vi "PromptUserWithDefault.vi"(7 "is Category?":bool, 9 "Recommended Name (\"\": None)":string, 10 "Structure Type":T1, 11 "Section":string) -> (1 "OK":bool, 2 "NewTag 2":string caption="NewTag")   [LabVIEW 2020]
uses:
  StructureTypes.ctl
  <userlib>/_OpenG.lib/appcontrol/appcontrol.llb/openg_application_control.lvlib
panel:
  in  "New Frame Name":string caption="NewTag"
  out "error out":errorcluster
  in  "error in (no error)":errorcluster
  out "String":string="Enter new case name or hit 'Cancel'."
  in  "Enable":bool=TRUE
  in  "Cancel":bool
  in  "OK2":bool
  in  "OK1":bool
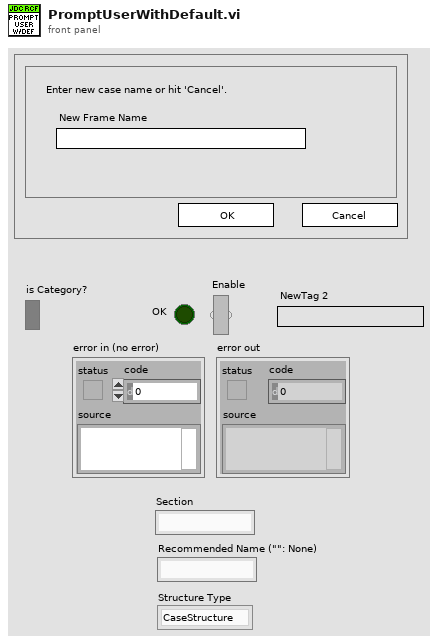
[diagram p1: front panel]
types:
  T1 = typedef "StructureTypes.ctl" = enum16{"CaseStructure", "EventStructure"}
  T2 = cluster{"Selection Start":u32, "Selection End":u32}
  T3 = cluster{"Input Name":string, "Input Data Type":i32}[]
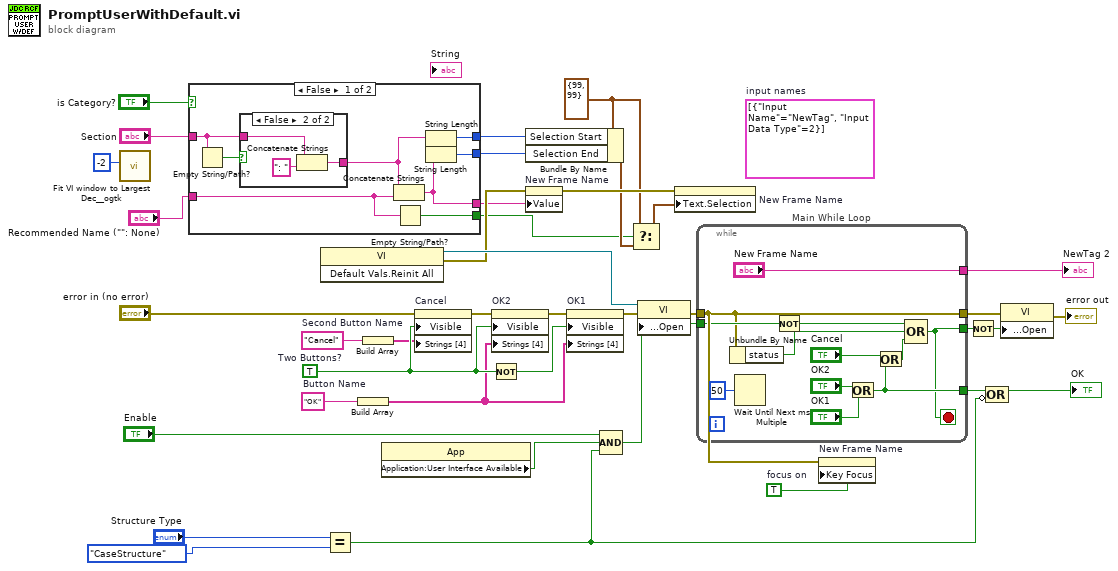
[diagram p0: block diagram]
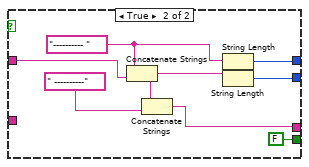
[diagram p3: hidden frame]
diagram:
  w6 = T2 {"Selection Start"=99, "Selection End"=99} ("Text.Selection")
  w23 = TRUE  # focus on
  (unwired) T3 [{"Input Name"="NewTag", "Input Data Type"=2}]  # input names
  w32 = "Cancel"  # Second Button Name
  w30 = "OK"  # Button Name
  w39 = TRUE  # Two Buttons?
  n1 = call <userlib>:"Fit VI window to Largest Dec__ogtk.vi"("border spacing (2 px)"=-2) -> ()  [unwired: 5 in, 2 out]
  n2 = case shown="False" "is Category?" {
    tunnel: "Section" -> [w41 w57]
    tunnel: "Recommended Name (\"\": None)" -> [w43 _]
    tunnel: [w46 w52] -> w7
    tunnel: [w45 w55] -> w4
    tunnel: [w44 w59] -> w3
    tunnel: [w42 FALSE] -> w1
    frame False {
      n3 = Empty String/Path?(string/path=w41) -> (empty?=w40:bool)
      n4 = case shown="False" w40 {
        tunnel: [w48 w50] -> w47
        tunnel: w41 -> [w48 w49]
        frame True {
        }
        frame False {
          n5 = Concatenate Strings(w49, ": " ("string")) -> (w50:string)
        }
      }
      n6 = Concatenate Strings(w47, w43) -> (w46:string)
      n7 = Empty String/Path?(string/path=w43) -> (empty?=w42:bool)
      n8 = String Length(string=w47) -> (length=w45:i32)
      n9 = String Length(string=w46) -> (length=w44:i32)
    }
    frame True {
      w54 = "---------- " ("Section")
      n10 = Concatenate Strings(w54, w57) -> (w53:string)
      n11 = Concatenate Strings(w53, " ----------" ("Section")) -> (w52:string)
      n12 = String Length(string=w54) -> (length=w55:i32)
      n13 = String Length(string=w53) -> (length=w59:i32)
    }
  }
  n14 = invoke class="VI" method="Default Vals.Reinit All"() -> (reference out=w24:refnum<vi>, error out=w16:errorcluster)  [unwired: 3 in, 1 out]
  n15 = Equal?(x="Structure Type", y=StructureTypes."CaseStructure") -> (x = y?=w11:bool)
  n16 = Build Array(w30) -> (w31:string[])
  n17 = Build Array(w32) -> (w33:string[])
  n18 = property class="App"() -> ("Application:User Interface Available"=w25:bool)  [unwired: 2 in, 2 out]
  n19 = property on="Cancel" class="Bool"(error in="error in (no error)", "Visible"=w39, "Strings [4]"=w33) -> (error out=w37:errorcluster)  [unwired: 1 in, 1 out]
  n20 = Not(x=w39) -> (.not. x?=w38:bool)
  n21 = property on="OK2" class="Bool"(error in=w37, "Visible"=w39, "Strings [4]"=w31) -> (error out=w36:errorcluster)  [unwired: 1 in, 1 out]
  n22 = Bundle By Name(cluster=w6, "Selection Start"=w4, "Selection End"=w3) -> (w5:T2)
  n23 = property on="New Frame Name" class="Str"(error in=w16, "Value"=w7) -> (error out=w15:errorcluster)  [unwired: 1 in, 1 out]
  n24 = property on="OK1" class="Bool"(error in=w36, "Visible"=w38, "Strings [4]"=w31) -> (error out=w29:errorcluster)  [unwired: 1 in, 1 out]
  n25 = Compound Arithmetic op=AND("Enable", w25, w11) -> (w26:bool)
  n26 = Select(t=w6, s=w1, f=w5) -> (s? t:f=w8:T2)
  n27 = property class="VI"(reference=w24, error in=w29, "Front Panel Window:Open"=w26) -> (error out=w28:errorcluster)  [unwired: 1 out]
  n28 = property on="New Frame Name" class="Str"(error in=w15, "Text.Selection"=w8) -> ()  [unwired: 1 in, 2 out]
  n29 = while "Main While Loop" {
    tunnel: [w70] -> w20
    tunnel: w26 -> [w69]
    tunnel: [w67] -> w34
    tunnel: w28 -> [w66]
    tunnel: [w66] -> w27
    tunnel: ["New Frame Name"] -> w18
    stop <- w67 stop-if-true
    n30 = Unbundle By Name(w66) -> ("status"=w64:bool)
    n31 = Wait Until Next ms Multiple(millisecond multiple=u32 50) -> ()  [unwired: 1 out]
    n32 = Not(x=w69) -> (.not. x?=w68:bool)
    n33 = Or(x="OK2", y="OK1") -> (x .or. y?=w70:bool)
    n34 = Or(x="Cancel", y=w70) -> (x .or. y?=w65:bool)
    n35 = Compound Arithmetic op=OR(w68, w64, w65) -> (w67:bool)
  }
  "NewTag 2" <- w18
  n36 = property on="New Frame Name" class="Str"(error in=w28, "Key Focus"=w23) -> ()  [unwired: 1 in, 2 out]
  n37 = Not(x=w34) -> (.not. x?=w35:bool)
  n38 = Compound Arithmetic op=OR(w20, invert w11) -> (→"OK":bool)
  n39 = property class="VI"(error in=w27, "Front Panel Window:Open"=w35) -> (error out=→"error out":errorcluster)  [unwired: 1 in, 1 out]
